vi "scada.vi"() -> ()   [LabVIEW 2014]
panel:
  out "SYSTEM-ON":bool
  out "SYSTEM-OFF":bool
  out "RIGHT":bool
  out "LEFT":bool
  out "STANJE":string
  out "FAULT":bool
  out "EMERGENCY-OFF":bool
  out "CENTER":bool
  in  "stop":bool
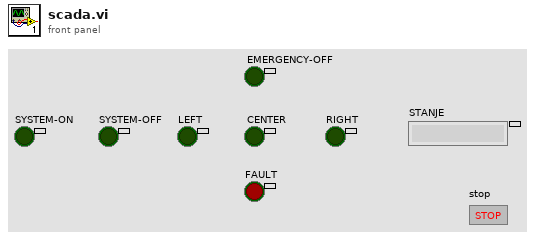
[diagram p1: front panel]
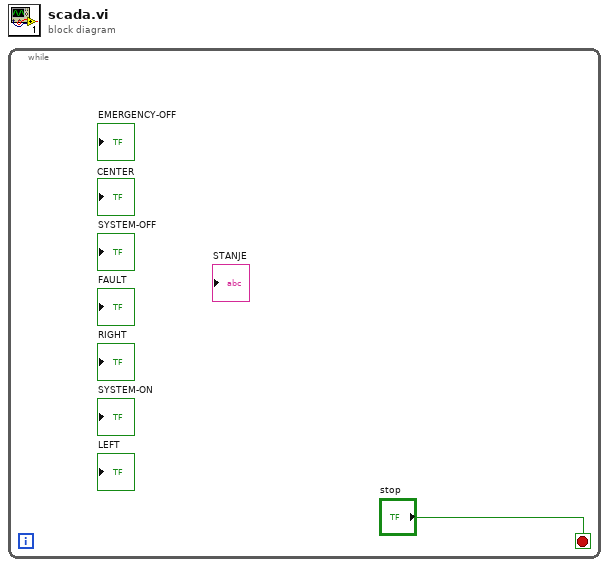
[diagram p0: block diagram]
diagram:
  n1 = while {
    stop <- "stop" stop-if-true
  }
